vi "to_json.vi"(8 "error in":errorcluster, 11 "workspace in":refnum<class "workspace.lvclass">) -> (0 "error out":errorcluster, 2 "json":string, 3 "workspace out":refnum<class "workspace.lvclass">, 4 "Not Default":bool)   [LabVIEW 2020, in "nominal types.lvlib" / "workspace.lvclass"]
uses:
  workspace.lvclass
  workspace.lvclass/workspace.ctl
  7c3b87de-daf8-40fc-939e-4f9244e9a4d8.vi
  bf7b01e1-8110-4372-be0e-405f04d60bdb.vi
  <vilib>/JDP Science/JSONtext/Variant to JSON Text.vi
  <vilib>/JDP Science/JSONtext/LVClass Serializer/JSONtext LVClass Serializer.lvclass
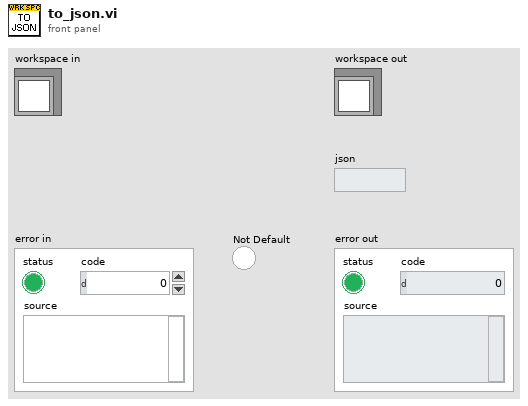
[diagram p1: front panel]
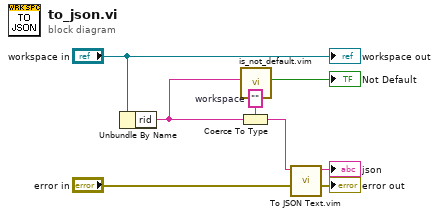
[diagram p0: block diagram]
diagram:
  w7 = ""  # workspace
  n1 = Unbundle By Name("workspace in") -> ("rid"=w2:string)
  n2 = Coerce To Type(0:w2, 1:w7) -> (2:w6:string)
  n3 = call "is_not_default.vim"("data"=w2) -> ("Not Default"=→"Not Default":bool)  [unwired: 10 in]
  n4 = call "To JSON Text.vim"("error in (no error)"="error in", "Anything"=w6) -> ("error out"=→"error out":errorcluster, "<JSON>"=→"json":string)  [unwired: 8 in]
  "workspace out" <- "workspace in"
